vi "ce exmpl - replace double asterisks .vi"(4 "formula in":string) -> (1 "formula out":string)   [LabVIEW 2021]
doc: "::: CalcExpress Toolkit :::\nCopyright (c) 2000-2026 Konstantin Shifershteyn. All rights reserved."
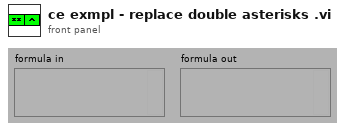
[diagram p1: front panel]
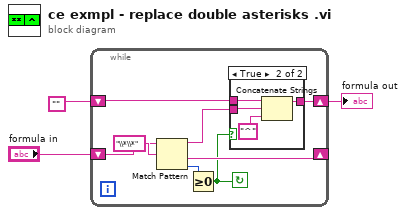
[diagram p0: block diagram]
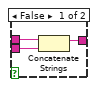
[diagram p2: hidden frame]
diagram:
  n1 = while {
    shift-left: "" -> [w6]
    shift-right: [w4] -> w1
    shift-left: "formula in" -> [w10]
    shift-right: [w9] -> _
    stop <- w7 continue-if-true
    n2 = Match Pattern(string=w10, regular expression="\\*\\*") -> (before substring=w5:string, after substring=w9:string, offset past match=w8:i32)  [unwired: 1 in, 1 out]
    n3 = Greater Or Equal To 0?(x=w8) -> (x >= 0?=w7:bool)
    n4 = case shown="True" w7 {
      tunnel: w6 -> [w14 w18]
      tunnel: w5 -> [w12 w16]
      tunnel: [w13 w17] -> w4
      frame False {
        n5 = Concatenate Strings(w14, w12) -> (w13:string)
      }
      frame True {
        n6 = Concatenate Strings(w18, w16, "^") -> (w17:string)
      }
    }
  }
  "formula out" <- w1
